vi "VIH Utility - MENU - Item Disabled Flag.vi"(11 "Disable?":bool) -> (3 "Disable flag":string)   [LabVIEW 2014]
doc: "::: VI Helpeks :::\nCopyright (c) 2000-2026 Konstantin Shifershteyn. All rights reserved."
panel:
  # "VI Helpeks\nCopyright (c) 2012-2026 Konstantin Shifershteyn"
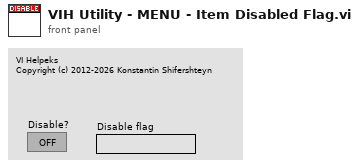
[diagram p1: front panel]
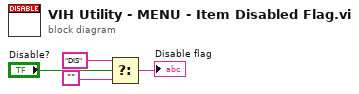
[diagram p0: block diagram]
diagram:
  n1 = Select(t="DIS", s="Disable?", f="") -> (s? t:f=→"Disable flag":string)
